vi "VIH Utility - MENU - Create Menu (Descriptors).vi"(8 "error in":errorcluster, 10 "Item Descriptors":T1[](array[typedef]), 11 "menu":refnum<k9>) -> (0 "error out":errorcluster, 3 "dup menu":refnum<k9>)   [LabVIEW 2014]
doc: "::: VI Helpeks :::\nCopyright (c) 2000-2026 Konstantin Shifershteyn. All rights reserved."
uses:
  VIH Utility - MENU - Menu Item Descriptor.ctl
  VIH Utility - MENU - Menu Item Type.ctl
panel:
  # "VI Helpeks\nCopyright (c) 2012-2026 Konstantin Shifershteyn"
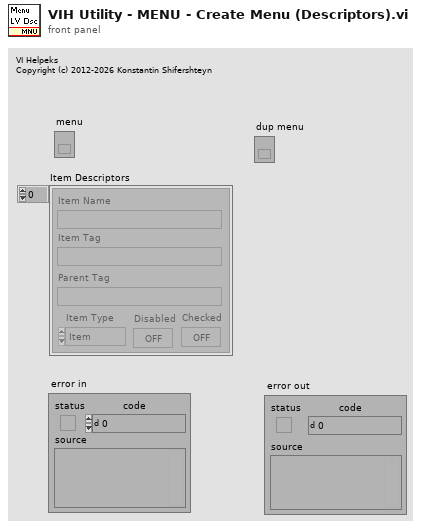
[diagram p1: front panel]
types:
  T1 = typedef "VIH Utility - MENU - Menu Item Descriptor.ctl" = cluster{"Item Name":string, "Item Tag":string, "Parent Tag":string, "Item Type":T2, "Disabled":bool, "Checked":bool}
  T2 = typedef "VIH Utility - MENU - Menu Item Type.ctl" = enum32{"Item", "SubMenu", "Separator"}
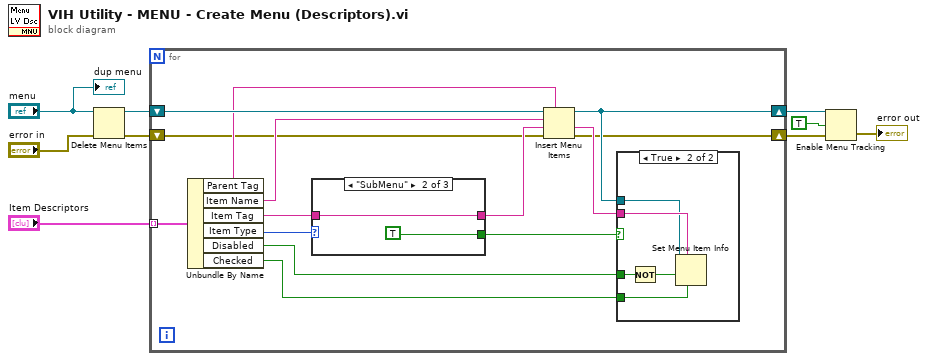
[diagram p0: block diagram]
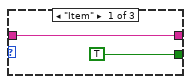
[diagram p3: hidden frame]
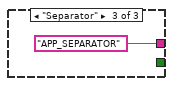
[diagram p4: hidden frame]
diagram:
  n1 = Delete Menu Items(6:"error in", 9:"menu") -> (0:w6:errorcluster, 3:w9:refnum<k9>)  [unwired: 2 out]
  n2 = for {
    tunnel: "Item Descriptors" -> [w23] mode=indexing
    shift-right: [w12] -> w8
    shift-left: w9 -> [w21]
    shift-right: [w10] -> w5
    shift-left: w6 -> [w11]
    n3 = Unbundle By Name(w23) -> ("Parent Tag"=w19:string, "Item Name"=w20:string, "Item Tag"=w18:string, "Item Type"=w22:T2, "Disabled"=w14:bool, "Checked"=w13:bool)
    n4 = case shown="\"SubMenu\"" w22 {
      tunnel: w18 -> [w30 w32 _]
      tunnel: [w30 w32 "APP_SEPARATOR" ("Item Tag")] -> w17
      tunnel: [TRUE TRUE _] -> w15
      frame "Item" {
      }
      frame "SubMenu" {
      }
      frame "Separator" {
      }
    }
    n5 = Insert Menu Items(5:w19, 6:w11, 7:w17, 8:w20, 9:w21) -> (0:w10:errorcluster, 1:w16:string, 3:w12:refnum<k9>)  [unwired: 1 out]
    n6 = case shown="True" w15 {
      tunnel: w16 -> [_ w28]
      tunnel: w12 -> [_ w27]
      tunnel: w14 -> [_ w26]
      tunnel: w13 -> [_ w24]
      frame False {
      }
      frame True {
        n7 = Not(x=w26) -> (.not. x?=w25:bool)
        n8 = Set Menu Item Info(6:w24, 7:w28, 9:w25, 11:w27) -> ()  [unwired: 2 in, 3 out]
      }
    }
  }
  n9 = Enable Menu Tracking(2:w5, 3:TRUE ("enable (T)"), 4:w8) -> (0:→"error out":errorcluster)  [unwired: 1 out]
  "dup menu" <- "menu"
